vi "mupEvalMulti.vi"(8 "error in (no error)":errorcluster, 11 "hParser in":u64) -> (0 "error out":errorcluster, 1 "nNum":i32, 2 "results":dbl[](array[numeric]), 3 "hParser out":u64)   [LabVIEW 2018, in "mupLib.lvlib"]
doc: "Evaluate all expressions. Returns the array of results. One result per expression."
uses:
  mupLib.lvlib
  <vilib>/Utility/error.llb/Error Cluster From Error Code.vi
  libmuparser-lv.dll
panel:
  # "Evaluate all expressions. Returns the array of results.\nOne result per expression."
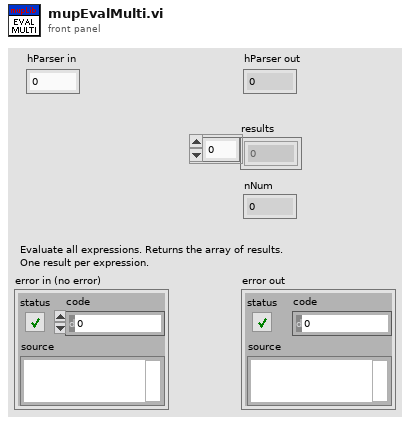
[diagram p1: front panel]
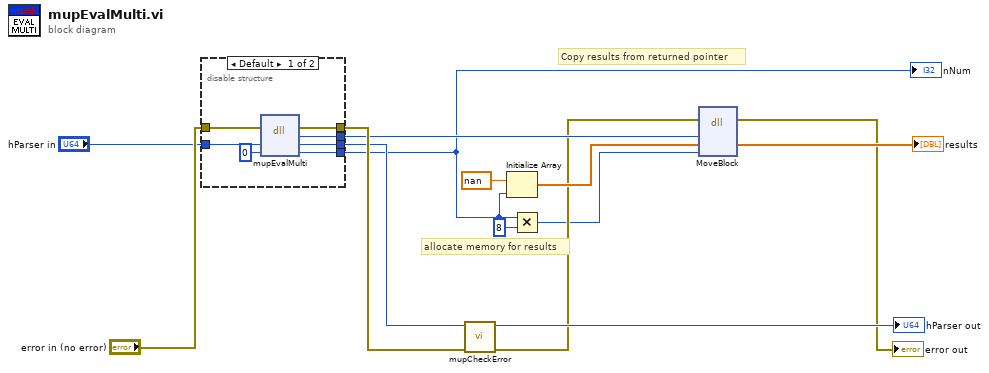
[diagram p0: block diagram]
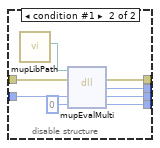
[diagram p2: hidden frame]
diagram:
  # "allocate memory for results"
  # "Copy results from returned pointer"
  n1 = disable-structure shown="Default" {
    disable-tunnel: [w21 w29] -> w14
    disable-tunnel: "error in (no error)" -> [w20 w28]
    disable-tunnel: "hParser in" -> [w19 w27]
    disable-tunnel: [w18 w26] -> w10
    disable-tunnel: [w16 w24] -> w7
    disable-tunnel: [w15 w23] -> w2
    frame condition #0 (active) {
      n2 = dll-call lib="C:/Users/leonidas/Documents/GitHub/LV-muParser/mupLib/libmuparser-lv.dll" fn="mupEvalMulti"(error in=w20, "hParser"=w19, "nNum"=0) -> (error out=w21:errorcluster, "return type"=w16:u64, "hParser"=w18:u64, "nNum"=w15:i32)  [unwired: 2 in, 1 out]
    }
    frame condition #1 {
      n3 = call "mupLibPath.vi"() -> ("libmuparser path"=w22:path)  [unwired: 11 in]
      n4 = dll-call lib="C:/Users/leonidas/Documents/GitHub/LV-muParser/mupLib/libmuparser-lv.dll" fn="mupEvalMulti"(path in=w22, error in=w28, "hParser"=w27, "nNum"=0) -> (error out=w29:errorcluster, "return type"=w24:u64, "hParser"=w26:u64, "nNum"=w23:i32)  [unwired: 1 in, 1 out]
    }
  }
  "nNum" <- w2
  n5 = call "mupCheckError.vi"("error in (no error)"=w14, "hParser in"=w10) -> ("error out"=w5:errorcluster, "hParser out"=→"hParser out":u64)  [unwired: 8 in]
  n6 = Initialize Array(nan ("element"), w2) -> (w8:dbl[])
  n7 = Multiply(x=w2, y=8) -> (x*y=w3:i32)
  n8 = dll-call lib="LabVIEW" fn="MoveBlock"(error in=w5, "ps"=w7, "pd"=w8, "size"=w3) -> (error out=→"error out":errorcluster, "pd"=→"results":dbl[])  [unwired: 5 in, 1 out]
